vi "Initialization VI.vi"(8 "error in (no error)":errorcluster, 10 "Custom XML":string, 11 "Device Item Ref in":T1 format="%.0x") -> (0 "error out":errorcluster, 3 "Device Item Ref out":T1 format="%.0x")   [LabVIEW 2025, in "Keithley-DAQ6510 System Explorer.lvlib"]
uses:
  Keithley-DAQ6510 System Explorer.lvlib
  <vilib>/NI VeriStand/Custom Device API/Custom Device Item Ref.ctl
  <vilib>/NI VeriStand/Custom Device API/Custom Device Channel.ctl
  <vilib>/NI VeriStand/Custom Device API/Custom Device Channel Type.ctl
  <vilib>/NI VeriStand/Custom Device API/Custom Device Waveform.ctl
  <vilib>/NI VeriStand/Custom Device API/Custom Device Waveform DataType.ctl
  <vilib>/NI VeriStand/Custom Device API/Set Item Property (Variant).vi
  <vilib>/NI VeriStand/Custom Device API/Custom Device API.lvlib
  Sys_DAQ_Global.vi
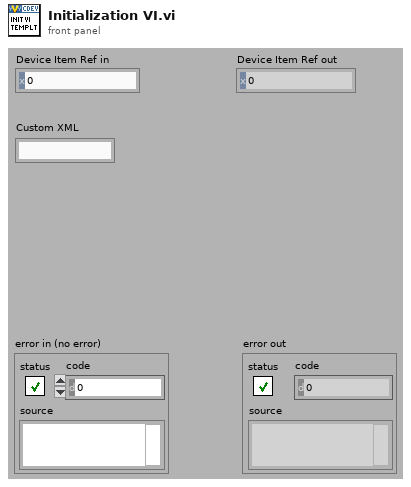
[diagram p1: front panel]
types:
  T1 = typedef "Custom Device API.lvlib/Custom Device Item Ref.ctl" = u64
  T2 = typedef "Custom Device API.lvlib/Custom Device Waveform.ctl" = cluster{"Data Type":T3, "Units":string}
  T3 = typedef "Custom Device API.lvlib/Custom Device Waveform DataType.ctl" = enum16{"Double", "Complex Double"}
  T4 = typedef "Custom Device API.lvlib/Custom Device Channel Type.ctl" = enum16{"Input", "Output"}
  T5 = typedef "Custom Device API.lvlib/Custom Device Channel.ctl" = cluster{"Type":T4, "Units":string, "Default Value":dbl, "Faultable":bool, "Scalable":bool}
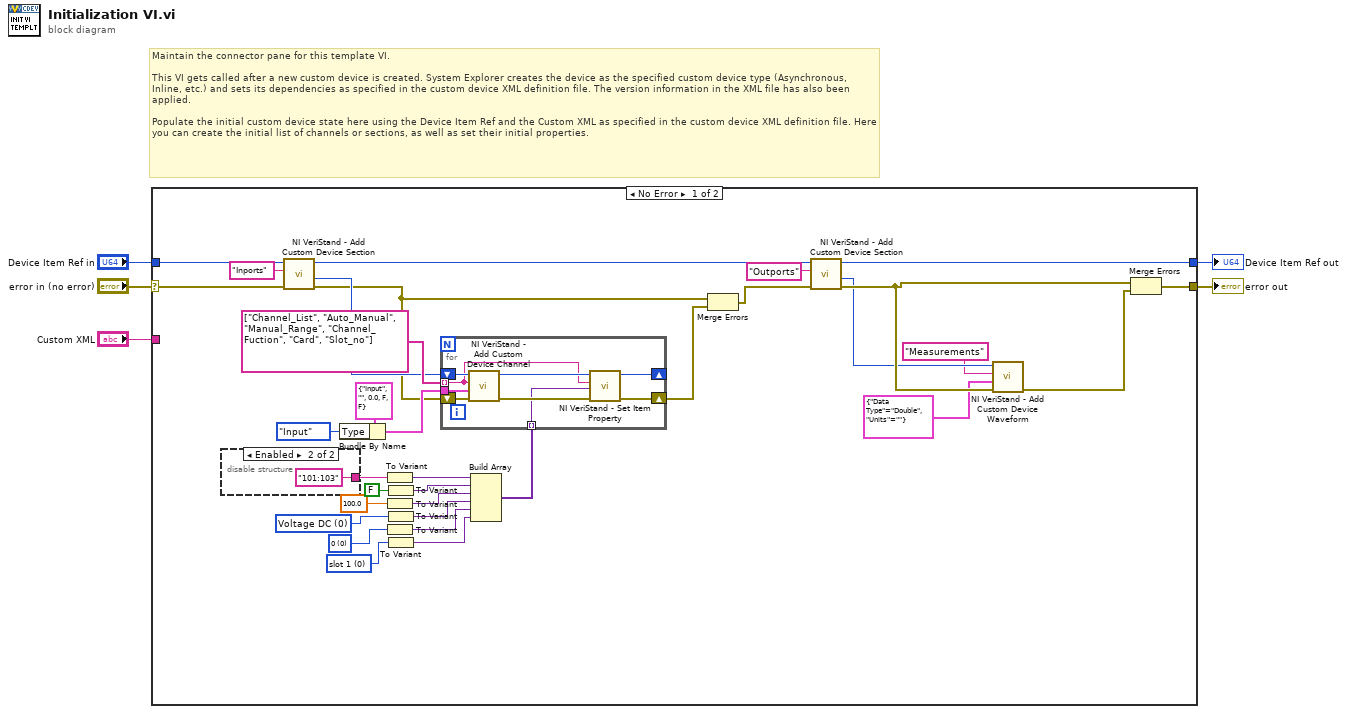
[diagram p0: block diagram]
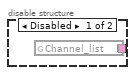
[diagram p2: hidden frame]
diagram:
  # "Maintain the connector pane for this template VI.\n\nThis VI gets called after a new custom device is created. System Explorer creates the device as the specified custom device type (Asynchronous, Inline, etc.) and sets its dependencies as specified in the custom device XML definition file. The version information in the XML file has also been applied.\n\nPopulate the initial custom device state here using the Device Item Ref and the Custom XML as specified in the custom device XML definition file. Here you can create the initial list of channels or sections, as well as set their initial properties."
  n1 = case shown="No Error" "error in (no error)" {
    selector: "error in (no error)" -> [w38 w51]
    tunnel: [w24 w51] -> w5
    tunnel: [w28 w50] -> w3
    tunnel: "Device Item Ref in" -> [w32 w50]
    tunnel: "Custom XML" -> [_ _]
    frame No Error {
      w13 = 0 items=["slot 1", "slot 2"] ("Slot Number (0: slot1)")
      w14 = 0 items=["0", "7700", "7701", "7702", "7703", "7705", "7706", "7707", "7708", "7709", "7710", "7711", "7712"] ("Pseudo Card (0:No pseudocard)")
      w15 = 0 items=["Voltage DC", "Voltage AC", "Current DC", "Current AC", "Resistance", "4-wire Resistance", "Diode", "Capacitance", "Temperature", "Continuity", "Frequency", "Period", "Voltage Ratio", "Digitize Voltage", "Digitize Current"] ("Function (0: Voltage DC)")
      n2 = disable-structure shown="Enabled" {
        disable-tunnel: [w39 "101:103" ("Channel_list")] -> w18
        frame Disabled {
          n3 = global read "Sys_DAQ_Global.vi" "Channel_list"() -> (w39:string)
        }
        frame Enabled {
        }
      }
      n4 = call <vilib>:"NI VeriStand - Add Custom Device Section.vi"("error in (no error)"=w38, "Section Name"="Inports", "Parent Ref in"=w32) -> ("error out"=w27:errorcluster, "Section Ptr"=w31:T1, "Parent Ref out"=w29:T1)  [unwired: 5 in, 1 out]
      n5 = Bundle By Name(cluster=T5 {"Type"=enum."Input", "Units"="", "Default Value"=0.0, "Faultable"=FALSE, "Scalable"=FALSE} ("Channel"), "Type"=Custom_Device_Channel_Type."Input") -> (w35:T5)
      n6 = To Variant(anything=w18) -> (Variant=w12:variant)
      n7 = To Variant(anything=100.0) -> (Variant=w10:variant)
      n8 = To Variant(anything=w14) -> (Variant=w8:variant)
      n9 = To Variant(anything=FALSE) -> (Variant=w11:variant)
      n10 = To Variant(anything=w15) -> (Variant=w9:variant)
      n11 = To Variant(anything=w13) -> (Variant=w7:variant)
      n12 = Build Array(w12, w11, w10, w9, w8, w7) -> (w6:variant[])
      n13 = for {
        tunnel: w35 -> [w48]
        tunnel: string[] ["Channel_List", "Auto_Manual", "Manual_Range", "Channel_Fuction", "Card", "Slot_no"] ("Channel Name") -> [w41] mode=indexing
        shift-right: [w43] -> w26
        shift-left: w27 -> [w49]
        shift-right: [w45] -> _
        shift-left: w31 -> [w47]
        tunnel: w6 -> [w42] mode=indexing
        n14 = call <vilib>:"NI VeriStand - Add Custom Device Channel.vi"("error in (no error)"=w49, "Channel"=w48, "Channel Name"=w41, "Parent Ref in"=w47) -> ("error out"=w44:errorcluster, "Parent Ref out"=w46:T1)  [unwired: 4 in, 2 out]
        n15 = call-poly <vilib>:"NI VeriStand - Set Item Property.vi"("error in (no error)"=w44, "Value"=w42, "Property Name"=w41, "Item Ref in"=w46) -> ("error out"=w43:errorcluster, "Item Ref out"=w45:T1)  [unwired: 5 in, 1 out]
      }
      n16 = Merge Errors(w27, w26) -> (w25:errorcluster)
      n17 = call <vilib>:"NI VeriStand - Add Custom Device Section.vi"("error in (no error)"=w25, "Section Name"="Outports", "Parent Ref in"=w29) -> ("error out"=w22:errorcluster, "Section Ptr"=w21:T1, "Parent Ref out"=w28:T1)  [unwired: 5 in, 1 out]
      n18 = call <vilib>:"NI VeriStand - Add Custom Device Waveform.vi"("error in (no error)"=w22, "Waveform"=T2 {"Data Type"=enum."Double", "Units"=""}, "Waveform Name"="Measurements" ("Channel Name"), "Parent Ref in"=w21) -> ("error out"=w23:errorcluster)  [unwired: 4 in, 3 out]
      n19 = Merge Errors(w22, w23) -> (w24:errorcluster)
    }
    frame Error {
    }
  }
  "error out" <- w5
  "Device Item Ref out" <- w3
